vi "GDSAPI_Example_CreateMethods2.vi"() -> ()   [LabVIEW 2020]
uses:
  GDSAPI_SubVIs/GDSAPI_ClassProviderType.ctl
  ClassProviders/Common/CommonVIs/CommonVIs_AttributeType.ctl
  ClassProviders/Common/CommonVIs/CommonVIs_AttributeDataType.ctl
  ClassProviders/Common/String/GDSString_AccessScopeModifierType.ctl
  ClassProviders/Common/String/GDSString_MethodDescriptionType.ctl
  ClassProviders/Common/String/GDSString_ModifierType.ctl
  ClassProviders/Common/CommonVIs/CommonVIs_PropertyType.ctl
  GDSAPI_CreateClassType.ctl
  GDSAPI_SubVIs/GDSAPI_ClassTemplateType.ctl
panel:
  out "error out":errorcluster
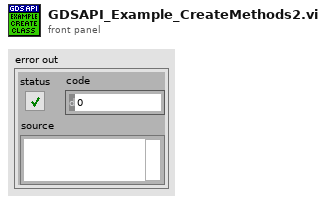
[diagram p1: front panel]
types:
  T1 = typedef "GDSString_MethodDescriptionType.ctl" = cluster{"ReturnType":T2, "MethodName":string, "AccessScope":T4, "Modifiers":T5[], "MethodDocumentation":string, "MethodContent":string, "MethodArguments":T2[], "GetProperty":T6, "SetProperty":T6}
  T2 = typedef "CommonVIs_AttributeType.ctl" = cluster{"Name":string, "DataType":T3, "ArrayDim":i32, "CtrlPath":path, "DataTypeString":string, "AccessScope":T4, "InitialData":variant}
  T3 = typedef "CommonVIs_AttributeDataType.ctl" = enum16{"UINT8", "INT8", "UINT16", "INT16", "UINT32", "INT32", "UINT64", "INT64", "SGL", "DBL", "EXT", "CSG", "CDB", "CXT", "TimeStamp", "STRING", "PATH", "BOOL", "ENUM", "RefNum", "VIRefNum", "LabVIEW Class", "Cluster", "Variant", "TypeDef", "Waveform", "LabVIEW Object", "Other", "void", "Set", "Map"}
  T4 = typedef "GDSString_AccessScopeModifierType.ctl" = enum16{"public", "private", "protected", "internal"}
  T5 = typedef "GDSString_ModifierType.ctl" = enum16{"abstract", "static", "final", "synchronized", "strictfp", "async", "const", "event", "extern", "new", "native ", "override", "partial", "readonly", "sealed", "unsafe", "virtual", "volatile"}
  T6 = typedef "CommonVIs_PropertyType.ctl" = cluster{"Active":bool, "AccessScope":T4, "Code":string}
  T7 = typedef "GDSAPI_ClassProviderType.ctl" = enum16{"LabVIEW Native(By value)", "GOOP-3(By reference)", "GOOP-4(By reference)"}
  T8 = typedef "GDSAPI_CreateClassType.ctl" = cluster{"ClassProvider":T7, "NewClassFolder":path, "ParentLvClassFilePath":path, "ClassName":string, "ClassDescription":string, "ClassTemplate":T9, "ParentInterfacesFilePath":path[]}
  T9 = typedef "GDSAPI_ClassTemplateType.ctl" = enum16{"Standard", "Singleton", "Interface(By Aggregation)", "Interface(By VI Server)"}
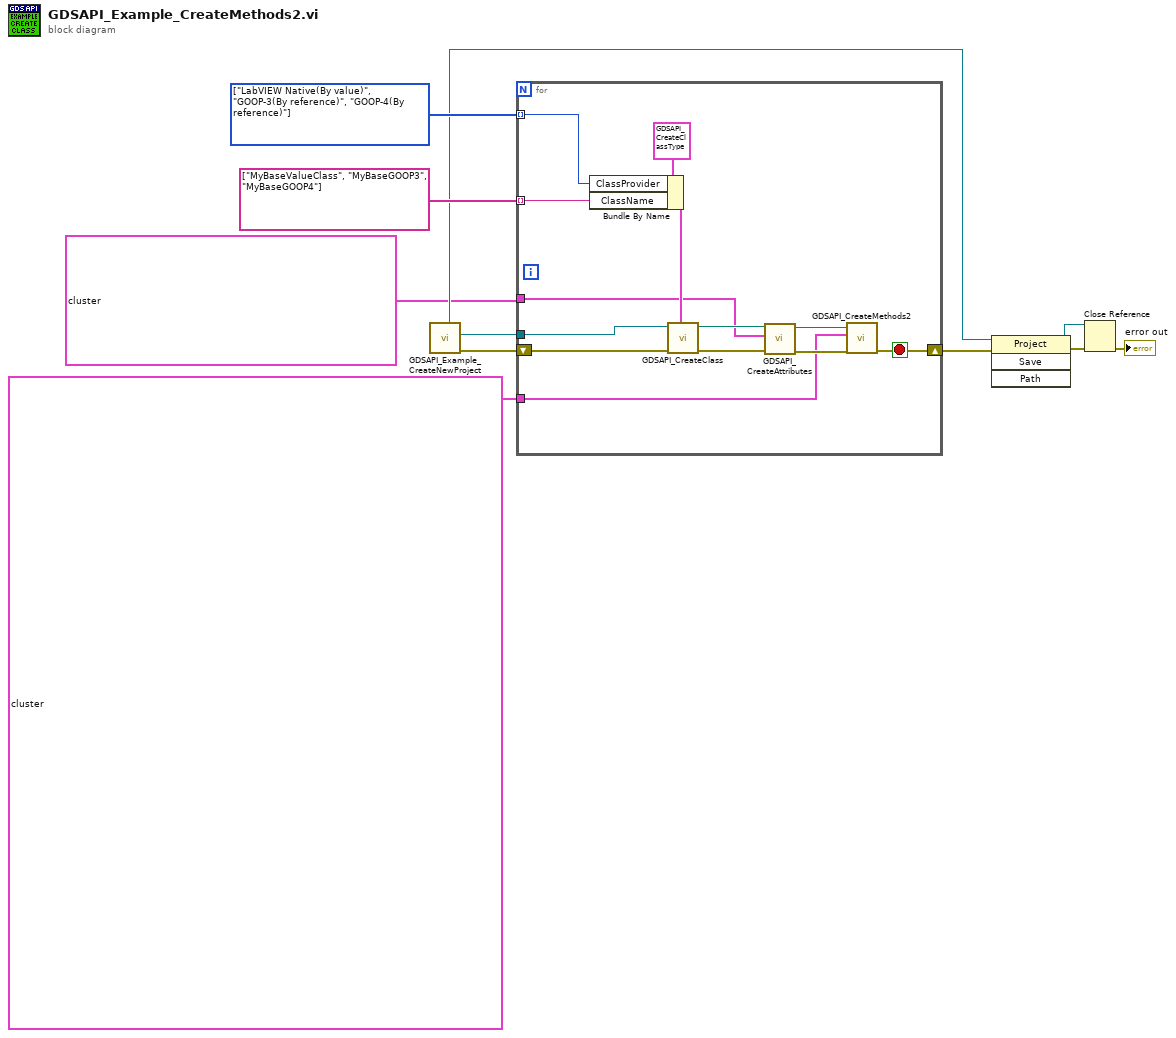
[diagram p0: block diagram]
diagram:
  w6 = T7[] [enum."LabVIEW Native(By value)", enum."GOOP-3(By reference)", enum."GOOP-4(By reference)"] items=["LabVIEW Native(By value)", "GOOP-3(By reference)", "GOOP-4(By reference)"]
  n1 = call "GDSAPI_Example_CreateNewProject.vi"() -> ("error out"=w11:errorcluster, "ProjectItem out"=w10:refnum<vi>, "ProjectRefOut"=w5:refnum<vi>)  [unwired: 8 in, 1 out]
  n2 = for {
    tunnel: w10 -> [w24]
    tunnel: string[] ["MyBaseValueClass", "MyBaseGOOP3", "MyBaseGOOP4"] -> [w22] mode=indexing
    tunnel: w6 -> [w21] mode=indexing
    shift-right: [w13] -> w3
    shift-left: w11 -> [w20]
    tunnel: T2[] [{"Name"="EmailsToSendTo", "DataType"=enum."STRING", "ArrayDim"=1, "CtrlPath"=path "", "DataTypeString"="", "AccessScope"=enum."public", "InitialData"=variant}, {"Name"="SmtpServer", "DataType"=enum."STRING", "ArrayDim"=0, "CtrlPath"=path "", "DataTypeString"="", "AccessScope"=enum."public", "InitialData"=variant}] ("Attributes") -> [w15]
    tunnel: T1[] [{"ReturnType"={"Name"="", "DataType"=enum."STRING", "ArrayDim"=1, "CtrlPath"=path "", "DataTypeString"="List<String>", "AccessScope"=enum."public", "InitialData"=variant(string "")}, "MethodName"="EmailsToSendTo", "AccessScope"=enum."public", "Modifiers"=[], "MethodDocumentation"="", "MethodContent"="public List<String> EmailsToSendTo { get; set; }", "MethodArguments"=[], "GetProperty"={"Active"=TRUE, "AccessScope"=enum."public", "Code"=""}, "SetProperty"={"Active"=TRUE, "AccessScope"=enum."public", "Code"=""}}, {"ReturnType"={"Name"="", "DataType"=enum."STRING", "ArrayDim"=0, "CtrlPath"=path "", "DataTypeString"="String", "AccessScope"=enum."public", "InitialData"=variant(string "")}, "MethodName"="SmtpServer", "AccessScope"=enum."public", "Modifiers"=[], "MethodDocumentation"="", "MethodContent"="public String SmtpServer { get; set; }", "MethodArguments"=[], "GetProperty"={"Active"=TRUE, "AccessScope"=enum."public", "Code"=""}, "SetProperty"={"Active"=TRUE, "AccessScope"=enum."public", "Code"=""}}, {"ReturnType"={"Name"="Sum", "DataType"=enum."DBL", "ArrayDim"=0, "CtrlPath"=path "", "DataTypeString"="", "AccessScope"=enum."public", "InitialData"=variant}, "MethodName"="Add Two Numbers", "AccessScope"=enum."public", "Modifiers"=[], "MethodDocumentation"="", "MethodContent"="Float X,Y,Sum;\nSum=X+Y;\n", "MethodArguments"=[{"Name"="X", "DataType"=enum."DBL", "ArrayDim"=0, "CtrlPath"=path "", "DataTypeString"="", "AccessScope"=enum."public", "InitialData"=variant}, {"Name"="Y", "DataType"=enum."DBL", "ArrayDim"=0, "CtrlPath"=path "", "DataTypeString"="", "AccessScope"=enum."public", "InitialData"=variant}], "GetProperty"={"Active"=FALSE, "AccessScope"=enum."public", "Code"=""}, "SetProperty"={"Active"=FALSE, "AccessScope"=enum."public", "Code"=""}}] ("Methods") -> [w14]
    stop <- w13 stop-if-true
    n3 = Bundle By Name(cluster=T8 {"ClassProvider"=enum."LabVIEW Native(By value)", "NewClassFolder"=path "", "ParentLvClassFilePath"=path "", "ClassName"="", "ClassDescription"="", "ClassTemplate"=enum."Standard", "ParentInterfacesFilePath"=[]} ("CreateClassType"), "ClassProvider"=w21, "ClassName"=w22) -> (w23:T8)
    n4 = call "GDSAPI_CreateClass.vi"("error in (no error)"=w20, "CreateClassType"=w23, "ProjectItemToCreateClassUnder"=w24) -> ("error out"=w19:errorcluster, "LvClassFileOut"=w17:path)  [unwired: 6 in, 1 out]
    n5 = call "GDSAPI_CreateAttributes.vi"("error in (no error)"=w19, "Attributes"=w15, "ClassPath(*.lvclass)"=w17) -> ("error out"=w18:errorcluster, "ClassPathOut(*.lvclass)"=w16:path)  [unwired: 7 in]
    n6 = call "GDSAPI_CreateMethods2.vi"("error in (no error)"=w18, "Methods"=w14, "ClassPath(*.lvclass)"=w16) -> ("error out"=w13:errorcluster)  [unwired: 7 in, 1 out]
  }
  n7 = invoke class="Project" method="Save"(reference=w5, error in=w3) -> (reference out=w8:refnum<vi>, error out=w9:errorcluster)  [unwired: 2 in, 2 out]
  n8 = Close Reference(reference=w8, error in (no error)=w9) -> (error out=→"error out":errorcluster)
